vi "Send Message.vi"(6 "Custom Attributes":T1[](array[typedef]), 8 "error in (no error)":errorcluster, 9 "Delay Seconds":i32=-1, 10 "Message Body":string, 11 "SQS in":refnum<class "Queue.lvclass">) -> (0 "error out":errorcluster, 1 "MD5 of Body":string, 2 "Message ID":string, 3 "SQS out":refnum<class "Queue.lvclass">, 4 "MD5 of Custom Attributes":string)   [LabVIEW 2015, in "NI_AWS_SQS.lvlib" / "Queue.lvclass"]
doc: "Delivers a message to the specified queue.\n\nImportant\nA message can include only XML, JSON, and unformatted text. The following Unicode characters are allowed:\n#x9 | #xA | #xD | #x20 to #xD7FF | #xE000 to #xFFFD | #x10000 to #x10FFFF\nAny characters not included in this list will be rejected. For more information, see the W3C specification for characters."
uses:
  Queue.lvclass
  Custom Attribute.ctl
  Custom Attribute Type.ctl
  Core/HTTP Request/Name Value Pair.ctl
  Core/HTTP Request/Request Options.ctl
  Core/HTTP Request/Region handling.ctl
  Core/HTTP Request/URL formatting.ctl
  Queue.lvclass/Queue.ctl
  Read Account Number.vi
  Read Name.vi
  Core/HTTP Request/HTTP Request.lvclass
  XML Parsing/NI_XML Parsing.lvlib
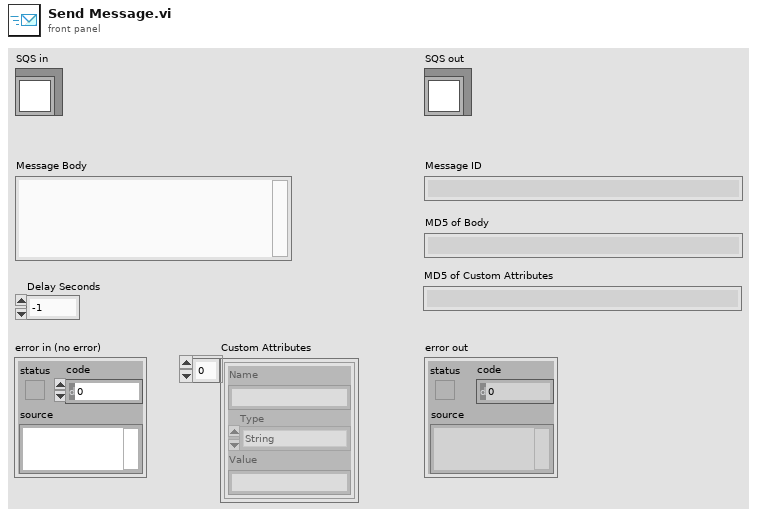
[diagram p1: front panel]
types:
  T1 = typedef "NI_AWS_SQS.lvlib/Queue.lvclass/Custom Attribute.ctl" = cluster{"Name":string, "Type":T2, "Value":string}
  T2 = typedef "NI_AWS_SQS.lvlib/Queue.lvclass/Custom Attribute Type.ctl" = enum16{"String", "Number", "Binary"}
  T3 = typedef "NI_AWS_Core.lvlib/HTTP Request.lvclass/Name Value Pair.ctl" = cluster{"name":string, "value":string}
  T4 = typedef "NI_AWS_Core.lvlib/HTTP Request.lvclass/Request Options.ctl" = cluster{"request headers":T3[], "request parameters":T3[], "request body":string, "region handling":T5, "URL formatting":T6}
  T5 = typedef "NI_AWS_Core.lvlib/HTTP Request.lvclass/Region handling.ctl" = enum16{"use region everywhere", "use region (authentication only)", "use region (URL only)", "ignore region everwhere"}
  T6 = typedef "NI_AWS_Core.lvlib/HTTP Request.lvclass/URL formatting.ctl" = enum16{"region-", "region."}
  T7 = typedef "NI_AWS_Core.lvlib/HTTP Request.lvclass/Response.ctl" = cluster{"Headers":string, "Body":string}
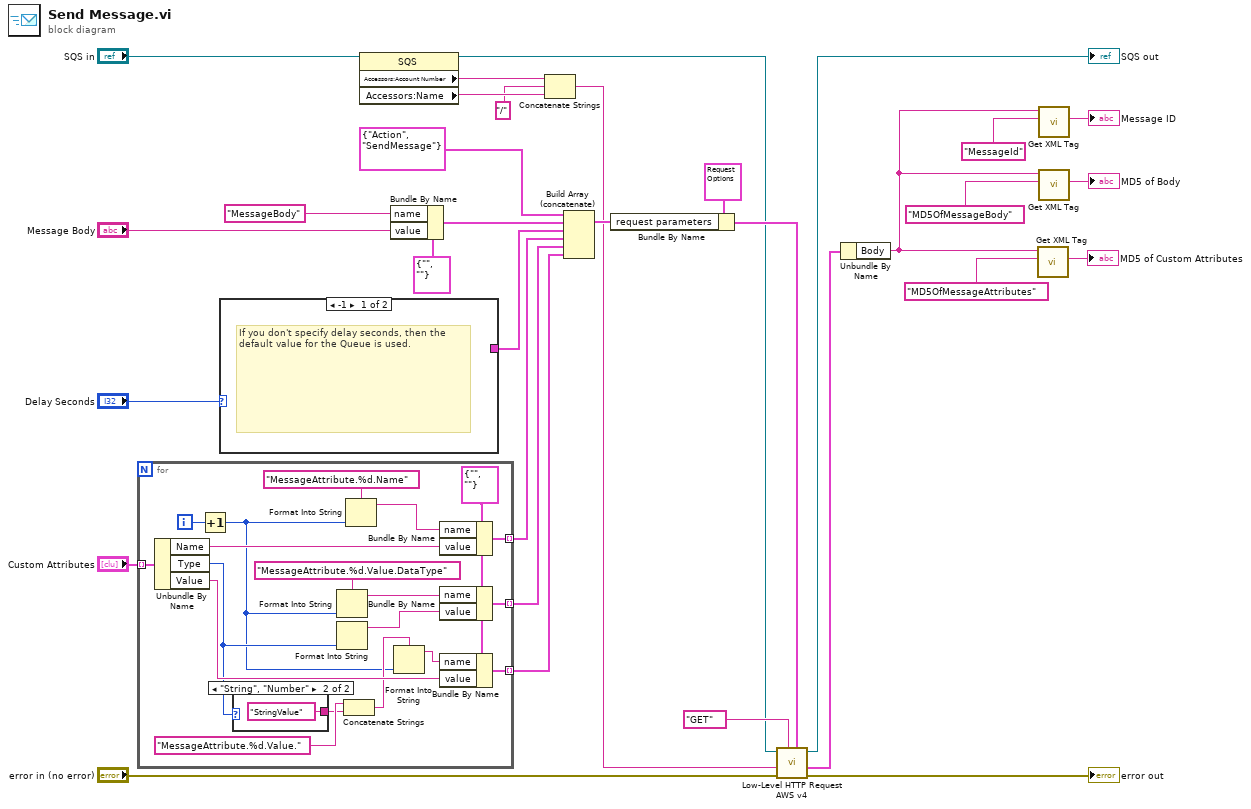
[diagram p0: block diagram]
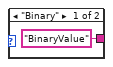
[diagram p2: hidden frame]
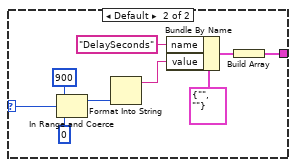
[diagram p3: hidden frame]
diagram:
  n1 = for {
    tunnel: "Custom Attributes" -> [w51] mode=indexing
    tunnel: [w49] -> w8 mode=indexing
    tunnel: [w48] -> w7 mode=indexing
    tunnel: [w47] -> w6 mode=indexing
    i -> [w39]
    w50 = T3 {"name"="", "value"=""} ("element")
    n2 = Unbundle By Name(w51) -> ("Name"=w45:string, "Type"=w35:T2, "Value"=w40:string)
    n3 = Increment(x=w39) -> (x+1=w33:i32)
    n4 = case shown="\"String\", \"Number\"" w35 {
      tunnel: ["BinaryValue" "StringValue"] -> w34
      frame "Binary" {
      }
      frame "String", "Number" {
      }
    }
    n5 = Format Into String(format string="MessageAttribute.%d.Value.DataType", w33) -> (resulting string=w42:string)  [unwired: 2 in, 1 out]
    n6 = Format Into String(w35) -> (resulting string=w41:string)  [unwired: 3 in, 1 out]
    n7 = Concatenate Strings("MessageAttribute.%d.Value.", w34) -> (w37:string)
    n8 = Format Into String(format string="MessageAttribute.%d.Name", w33) -> (resulting string=w44:string)  [unwired: 2 in, 1 out]
    n9 = Format Into String(format string=w37, w33) -> (resulting string=w38:string)  [unwired: 2 in, 1 out]
    n10 = Bundle By Name(cluster=w50, "name"=w44, "value"=w45) -> (w49:T3)
    n11 = Bundle By Name(cluster=w50, "name"=w42, "value"=w41) -> (w48:T3)
    n12 = Bundle By Name(cluster=w50, "name"=w38, "value"=w40) -> (w47:T3)
  }
  n13 = case shown="-1" "Delay Seconds" {
    selector: "Delay Seconds" -> [_ w58]
    tunnel: [_ w54] -> w16
    frame -1 {
      # "If you don't specify delay seconds, then the default value for the Queue is used."
    }
    frame Default {
      n14 = In Range and Coerce(upper limit=900, x=w58, lower limit=0) -> (coerced(x)=w57:i32)  [unwired: 1 out]
      n15 = Format Into String(w57) -> (resulting string=w59:string)  [unwired: 3 in, 1 out]
      n16 = Bundle By Name(cluster=T3 {"name"="", "value"=""} ("element"), "name"="DelaySeconds", "value"=w59) -> (w61:T3)
      n17 = Build Array(w61) -> (w54:T3[])
    }
  }
  n18 = property class="SQS"(reference="SQS in") -> (reference out=w1:refnum<class "Queue.lvclass">, "Accessors:Account Number"=w27:string, "Accessors:Name"=w26:string)  [unwired: 1 in, 1 out]
  n19 = Bundle By Name(cluster=T3 {"name"="", "value"=""} ("element"), "name"="MessageBody", "value"="Message Body") -> (w17:T3)
  n20 = Concatenate Strings(w27, "/", w26) -> (w24:string)
  n21 = Build Array (concatenate)(T3 {"name"="Action", "value"="SendMessage"} ("Cluster"), w17, w16, w8, w7, w6) -> (w28:T3[])
  n22 = Bundle By Name(cluster=T4 {"request headers"=[], "request parameters"=[{"name"="Action", "value"="ListQueues"}], "request body"="", "region handling"=enum."use region everywhere", "URL formatting"=enum."region."} ("Request Options"), "request parameters"=w28) -> (w3:T4)
  n23 = call "Low-Level HTTP Request AWS v4.vi"("Request Options"=w3, "HTTP-Verb"="GET", "error in (no error)"="error in (no error)", "URL Suffix"=w24, "AWS Core in"=w1) -> ("error out"=→"error out":errorcluster, "Response"=w5:T7, "AWS Core out"=→"SQS out":refnum<class "Queue.lvclass">)  [unwired: 3 in, 1 out]
  n24 = Unbundle By Name(w5) -> ("Body"=w10:string)
  n25 = call "Get XML Tag.vi"("Tag name"="MD5OfMessageAttributes", "XML String in"=w10) -> ("Tag value"=→"MD5 of Custom Attributes":string)  [unwired: 5 in, 4 out]
  n26 = call "Get XML Tag.vi"("Tag name"="MessageId", "XML String in"=w10) -> ("Tag value"=→"Message ID":string)  [unwired: 5 in, 4 out]
  n27 = call "Get XML Tag.vi"("Tag name"="MD5OfMessageBody", "XML String in"=w10) -> ("Tag value"=→"MD5 of Body":string)  [unwired: 5 in, 4 out]
